vi "Test Helper Loop Broadcast Stopped on Error.vi"(8 "error in (no error)":errorcluster, 11 "Helper Loop Test In":refnum<class "Helper Loop Test.lvclass">) -> (0 "error out":errorcluster, 3 "Helper Loop Test Out":refnum<class "Helper Loop Test.lvclass">)   [LabVIEW 2020, in "Helper Loop Test.lvclass"]
uses:
  Helper Loop Test.lvclass
  C:/Program Files (x86)/National Instruments/LabVIEW 2020/vi.lib/Astemes/LUnit/Test Case.lvclass
  source/Framework Test Suite/Mock Process/Mock Process.lvclass
  C:/git/astemes-triarc-framework/source/Framework/Process/Process.lvclass
  source/Framework/Process/Process.lvclass/Process.ctl
  <vilib>/Astemes/LUnit/Test Case.lvclass/Test Case.ctl
  cf682f82-6362-4fa3-93a3-bc290b111215.vi
  source/Framework/Broadcast Event Dequeuers/Execution timer.vi
  source/Framework/Process/Private/SubVIs/Wait for finish.vi
  source/Framework/Process/Private/SubVIs/Set Lifecycle State.vi
  source/Framework/Process/Protected/Messaging/Send Message.vi
  <vilib>/Astemes/LUnit/Append Pass Result.vi
  <vilib>/Astemes/LUnit/Append Fail Result.vi
  cf682f82-6362-4fa3-93a3-bc290b111215.vi/9c5d11cd-9439-4240-a1ee-d9baace9c924.vi
  source/Framework/Process/Private/SubVIs/Handle Debug Data.vi
  <vilib>/Astemes/LUnit/Run In UI.vi
  source/Framework/Logging/Log Debug.vi
  <vilib>/AdvancedString/1D String Array to Delimited String.vi
  <vilib>/Utility/High Resolution Relative Seconds.vi
  <vilib>/Utility/error.llb/Clear Errors.vi
  source/Framework/Broadcast Event Dequeuers/Dequeue Broadcast Message.vi
  source/Framework/Process/Public/Lifecycle/Get Lifecycle State.vi
  <vilib>/Utility/error.llb/Error Cluster From Error Code.vi
  source/Framework/Process/Public/Read Name.vi
  source/Framework/Callback/Callback.lvclass
  source/Framework/Process/Process.lvclass
  Helper Loop Test.lvclass/Helper Loop Test.ctl
  source/Framework/Broadcast Event Dequeuers/Broadcast Event Dequeuers.lvlib
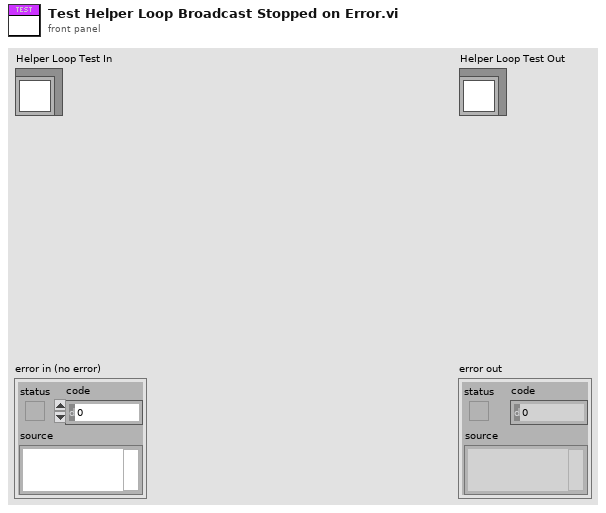
[diagram p1: front panel]
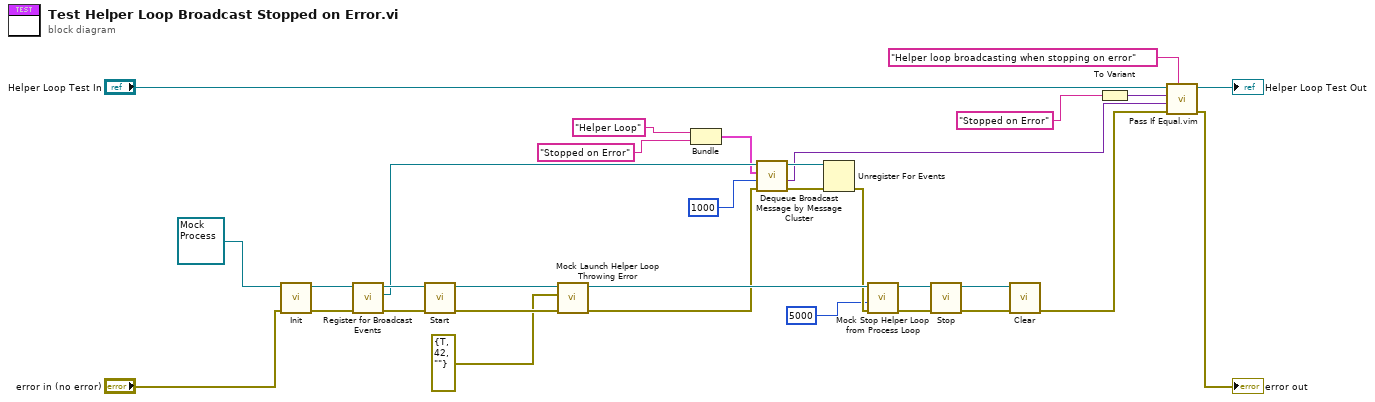
[diagram p0: block diagram]
diagram:
  n1 = call-dynamic "Init.vi"("error in (no error)"="error in (no error)", "Mock Process In"=refnum<class "Mock Process.lvclass"> refnum) -> ("error out"=w31:errorcluster, "Mock Process Out"=w32:refnum<class "Mock Process.lvclass">)  [unwired: 8 in]
  n2 = call "Register for Broadcast Events.vi"("error in (no error)"=w31, "Process In"=w32) -> ("error out"=w29:errorcluster, "Event Registration Refnum Out"=w16:refnum<event-registration>, "Process Out"=w30:refnum<class "Mock Process.lvclass">)  [unwired: 7 in]
  n3 = call "Start.vi"("error in (no error)"=w29, "Process In"=w30) -> ("error out"=w27:errorcluster, "Process Out"=w28:refnum<class "Mock Process.lvclass">)  [unwired: 7 in, 1 out]
  n4 = call "Mock Launch Helper Loop Throwing Error.vi"("error in (no error)"=w27, "Error message"=errorcluster {"status"=TRUE, "code"=42, "source"=""}, "Mock Process in"=w28) -> ("error out"=w14:errorcluster, "Mock Process out"=w26:refnum<class "Mock Process.lvclass">)  [unwired: 7 in]
  n5 = Bundle("y"="Helper Loop", "Description"="Stopped on Error") -> (w2:cluster{"y":string, "Description":string})  [unwired: 1 in]
  n6 = call "Dequeue Broadcast Message by Message Cluster.vi"("error in (no error)"=w14, "Timeout (-1)"=1000, "Message"=w2, "Event Registration Refnum"=w16) -> ("error out"=w8:errorcluster, "Message Data"=w7:variant, "Event Registration Refnum Out"=w10:refnum<event-registration>)  [unwired: 3 in, 2 out]
  n7 = Unregister For Events(event registration refnum=w10, error in=w8) -> (error out=w13:errorcluster)
  n8 = call "Mock Stop Helper Loop from Process Loop.vi"("error in (no error)"=w13, "timeout in ms (-1)"=5000, "Mock Process in"=w26) -> ("error out"=w24:errorcluster, "Mock Process out"=w25:refnum<class "Mock Process.lvclass">)  [unwired: 6 in, 1 out]
  n9 = call "Stop.vi"("error in (no error)"=w24, "Process In"=w25) -> ("error out"=w23:errorcluster, "Process Out"=w5:refnum<class "Mock Process.lvclass">)  [unwired: 7 in, 1 out]
  n10 = call-dynamic "Clear.vi"("error in (no error)"=w23, "Mock Process In"=w5) -> ("error out"=w22:errorcluster)  [unwired: 9 in]
  n11 = To Variant(anything="Stopped on Error" ("Description")) -> (Variant=w1:variant)
  n12 = call "Pass If Equal.vim"("Description"="Helper loop broadcasting when stopping on error", "error in (no error)"=w22, "Actual"=w7, "Expected"=w1, "LUnit Test Case In"="Helper Loop Test In") -> ("error out"=→"error out":errorcluster, "LUnit Test Case Out"=→"Helper Loop Test Out":refnum<class "Helper Loop Test.lvclass">)  [unwired: 5 in]
